vi "Remove Channel.vi"(8 "error in (no error)":errorcluster, 10 "AIO_CFG":refnum<class "AIO-Configuration.lvclass">, 11 "UI Template in":refnum<class "AIO_Panel.lvclass">) -> (0 "error out":errorcluster, 3 "UI Template out":refnum<class "AIO_Panel.lvclass">)   [LabVIEW 2021, in "Simulator-Channel.lvlib" / "AIO_Panel.lvlib" / "AIO_Panel.lvclass"]
uses:
  AIO_Panel.lvclass
  C:/Program Files/National Instruments/LabVIEW 2021/vi.lib/ActorFramework/Actor/Actor.lvclass
  Dependencies/AIO-Channel.lvlibp/Channels/AIO-Channel/AIO-Configuration_class/AIO-Configuration.lvclass
  C:/Users/averna/Documents/LV Gym DEMO/Factory Pattern/Device Channels/Dependencies/AIO-Channel.lvlibp/Generic Channel/Channel/Configuration_class/Configuration.lvclass
  AIO_Panel.lvclass/AIO_Panel.ctl
  <vilib>/ActorFramework/Actor/Actor.lvclass/Actor.ctl
  <vilib>/ActorFramework/Message Enqueuer/Message Enqueuer.lvclass/Message Enqueuer.ctl
  <vilib>/ActorFramework/Message Enqueuer/Init from Existing Queue.vi
  <vilib>/ActorFramework/Message Enqueuer/Enqueue.vi
  <vilib>/ActorFramework/Stop Msg/Stop Msg.lvclass
  C:/Program Files/National Instruments/LabVIEW 2021/vi.lib/ActorFramework/Message/Message.lvclass
  <vilib>/ActorFramework/Message Priority Queue/Priority Enqueue.vi
  <vilib>/ActorFramework/Message Enqueuer/Message Enqueuer.lvclass
  <vilib>/ActorFramework/Actor/Actor.lvclass
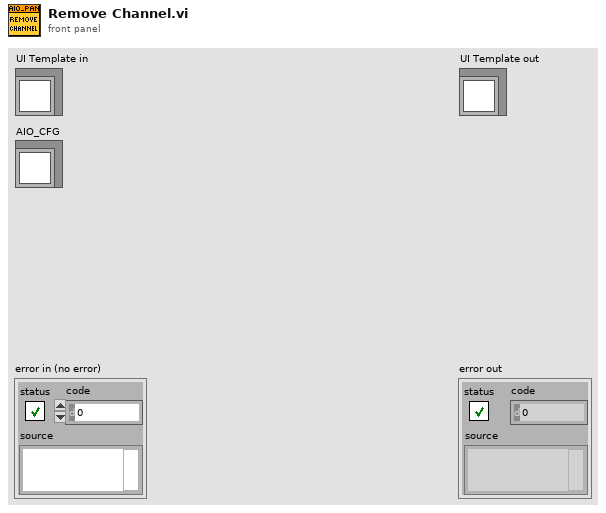
[diagram p1: front panel]
types:
  T1 = typedef "AIO-Channel.lvlibp/AIO-Configuration.lvclass/Direction.ctl" = enum16{"Input", "Output"}
  T2 = typedef "Simulator-Channel.lvlib/AIO_Panel.lvlib/AIO_Panel.lvclass/info.ctl" = cluster{"Name":string, "Numeric":dbl, "Unit":string}
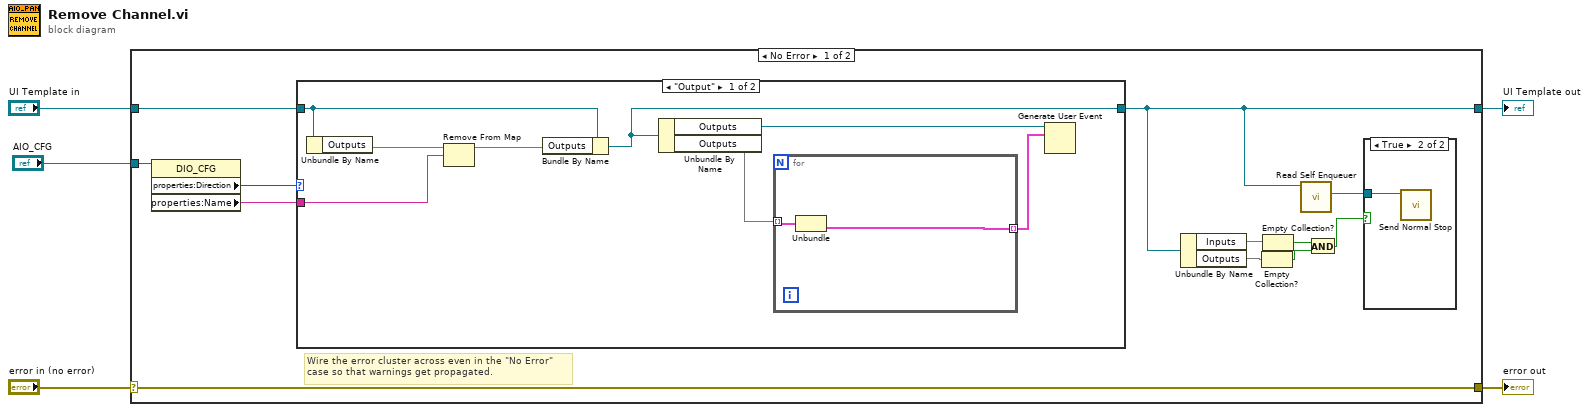
[diagram p0: block diagram]
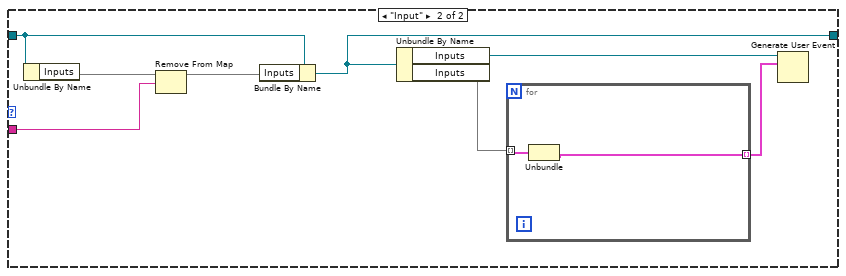
[diagram p3: hidden frame]
diagram:
  n1 = case shown="No Error" "error in (no error)" {
    selector: "error in (no error)" -> [w17 w40]
    tunnel: [w17 w40] -> w4
    tunnel: [w8 w39] -> w2
    tunnel: "UI Template in" -> [w15 w39]
    tunnel: "AIO_CFG" -> [w16 _]
    frame No Error {
      # "Wire the error cluster across even in the \"No Error\"\ncase so that warnings get propagated."
      n2 = property class="DIO_CFG"(reference=w16) -> ("properties:Direction"=w14:T1, "properties:Name"=w13:string)  [unwired: 1 in, 2 out]
      n3 = case shown="\"Output\"" w14 {
        tunnel: [w22 w29] -> w8
        tunnel: w15 -> [w26 w36]
        tunnel: w13 -> [w20 w33]
        frame "Output" {
          n4 = Unbundle By Name(w26) -> ("Outputs"=w21:map{string, T2})
          n5 = Remove From Map(10:w20, 11:w21) -> (3:w19:map{string, T2})  [unwired: 2 out]
          n6 = Bundle By Name(cluster=w26, "Outputs"=w19) -> (w22:refnum<class "AIO_Panel.lvclass">)
          n7 = Unbundle By Name(w22) -> ("Outputs"=w24:refnum<user-event>, "Outputs"=w25:map{string, T2})
          n8 = for {
            tunnel: w25 -> [w28] mode=indexing
            tunnel: [w27] -> w23 mode=indexing
            n9 = Unbundle(w28) -> ("Info"=w27:T2)  [unwired: 1 out]
          }
          n10 = Generate User Event(user event=w24, event data cluster=w23) -> ()  [unwired: 2 in, 2 out]
        }
        frame "Input" {
          n11 = Unbundle By Name(w36) -> ("Inputs"=w35:map{string, T2})
          n12 = Remove From Map(10:w33, 11:w35) -> (3:w34:map{string, T2})  [unwired: 2 out]
          n13 = Bundle By Name(cluster=w36, "Inputs"=w34) -> (w29:refnum<class "AIO_Panel.lvclass">)
          n14 = Unbundle By Name(w29) -> ("Inputs"=w31:refnum<user-event>, "Inputs"=w32:map{string, T2})
          n15 = for {
            tunnel: w32 -> [w38] mode=indexing
            tunnel: [w37] -> w30 mode=indexing
            n16 = Unbundle(w38) -> ("Info"=w37:T2)  [unwired: 1 out]
          }
          n17 = Generate User Event(user event=w31, event data cluster=w30) -> ()  [unwired: 2 in, 2 out]
        }
      }
      n18 = Unbundle By Name(w8) -> ("Inputs"=w12:map{string, T2}, "Outputs"=w11:map{string, T2})
      n19 = Empty Collection?(1:w11) -> (0:w9:bool)
      n20 = Empty Collection?(1:w12) -> (0:w10:bool)
      n21 = call <vilib>:"Read Self Enqueuer.vi"("Actor"=w8) -> ("Self Enqueuer"=w7:refnum<class "Message Enqueuer.lvclass">)  [unwired: 10 in]
      n22 = And(x=w10, y=w9) -> (x .and. y?=w6:bool)
      n23 = case shown="True" w6 {
        tunnel: w7 -> [_ w18]
        frame False {
        }
        frame True {
          n24 = call <vilib>:"Send Normal Stop.vi"("Message Enqueuer"=w18) -> ()  [unwired: 10 in, 1 out]
        }
      }
    }
    frame Error {
    }
  }
  "error out" <- w4
  "UI Template out" <- w2
